vi "Host_Sequence_Executor_GUI.vi"(4 "Configured Displacement SP (mm)":dbl=2.5, 5 "Configured Flow Setpoint (L/min)":dbl=45.0, 6 "Configured Pressure Tolerance (bar)":dbl=2.0, 7 "Configured Pressure Setpoint (bar)":dbl=100.0, 8 "error in (no error)":errorcluster={"status"=FALSE, "code"=0, "source"="\"\""}, 9 "Active Step Name":string="Step 1: 100 bar VTU Sweep", 10 "Active Step Index":i32=1, 11 "Execute Run (True to run)":bool=TRUE, 12 "Dwell Duration (ms)":i32=2000) -> (0 "error out":errorcluster, 1 "Step Execution Summary":string, 2 "Live Measured Flow (L/min)":dbl, 3 "Live Measured Pressure (bar)":dbl, 13 "Pump Power (kW)":dbl, 14 "Step Condition Met?":bool, 15 "Event Audit Log":string)   [LabVIEW 2026]
doc: "INTENT: Master Configuration & Execution GUI for Universal Sequence Executor, modeled after official NI Queued Message Handler and State Machine design patterns. Features interactive step sequence table, setpoint dispatch, real-time I/O monitoring, condition tolerance checking, and pass/fail summary."
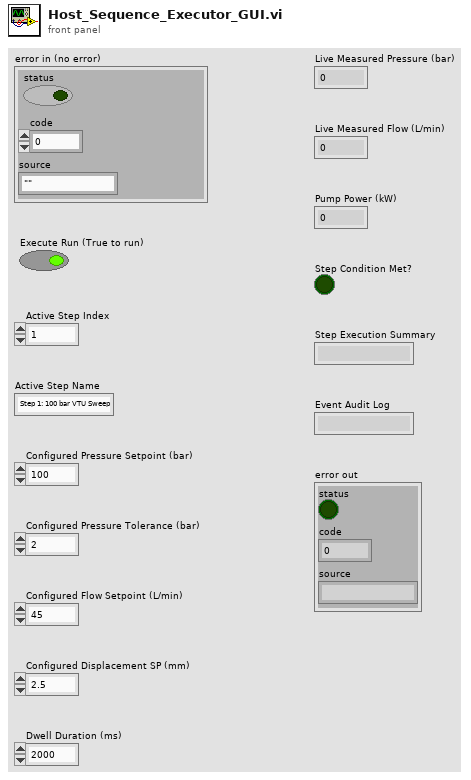
[diagram p1: front panel]
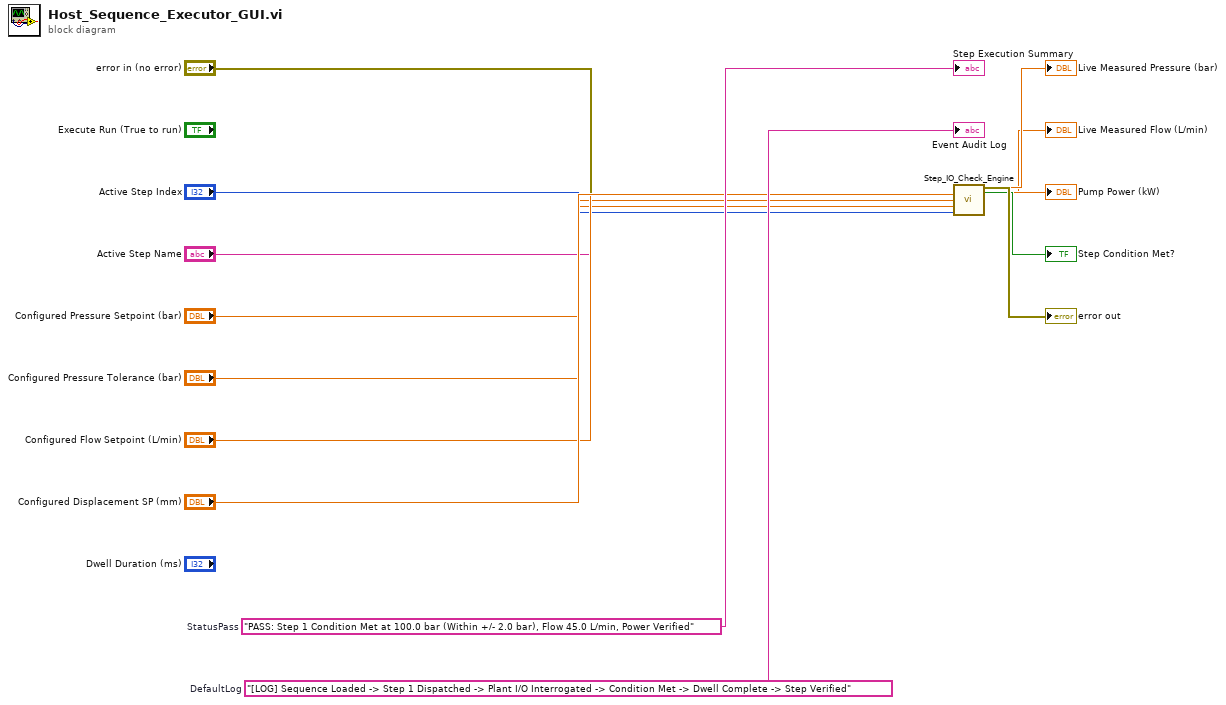
[diagram p0: block diagram]
diagram:
  w14 = "[LOG] Sequence Loaded -> Step 1 Dispatched -> Plant I/O Interrogated -> Condition Met -> Dwell Complete -> Step Verified"  # DefaultLog
  w13 = "PASS: Step 1 Condition Met at 100.0 bar (Within +/- 2.0 bar), Flow 45.0 L/min, Power Verified"  # StatusPass
  n1 = call "Step_IO_Check_Engine.vi"("Target Displacement SP (mm)"="Configured Displacement SP (mm)", "Target Flow SP (L/min)"="Configured Flow Setpoint (L/min)", "Tolerance (bar)"="Configured Pressure Tolerance (bar)", "error in (no error)"="error in (no error)", "Target Pressure SP (bar)"="Configured Pressure Setpoint (bar)", "Step Name"="Active Step Name", "Step No"="Active Step Index") -> ("error out"=→"error out":errorcluster, "Condition Met"=→"Step Condition Met?":bool, "Actual Power (kW)"=→"Pump Power (kW)":dbl, "Actual Flow (L/min)"=→"Live Measured Flow (L/min)":dbl, "Actual Pressure (bar)"=→"Live Measured Pressure (bar)":dbl)  [unwired: 4 in]
  "Step Execution Summary" <- w13
  "Event Audit Log" <- w14
